vi "Configure Secured TCP Client Certificate and Key.vi"(7 "Client X.509 Certificate":path, 8 "error in (no error)":errorcluster, 9 "password":string, 10 "Client Private Key":path, 11 "Connection.TCP-TLS in":refnum<class "Connection.TCP-TLS.lvclass">) -> (0 "error out":errorcluster, 2 "Auth Client?":bool, 3 "Connection.TCP-TLS out":refnum<class "Connection.TCP-TLS.lvclass">)   [LabVIEW 2020, in "Connection.TCP-TLS.lvclass"]
uses:
  Connection.TCP-TLS.lvclass
  Connection.TCP-TLS.lvclass/Connection.TCP-TLS.ctl
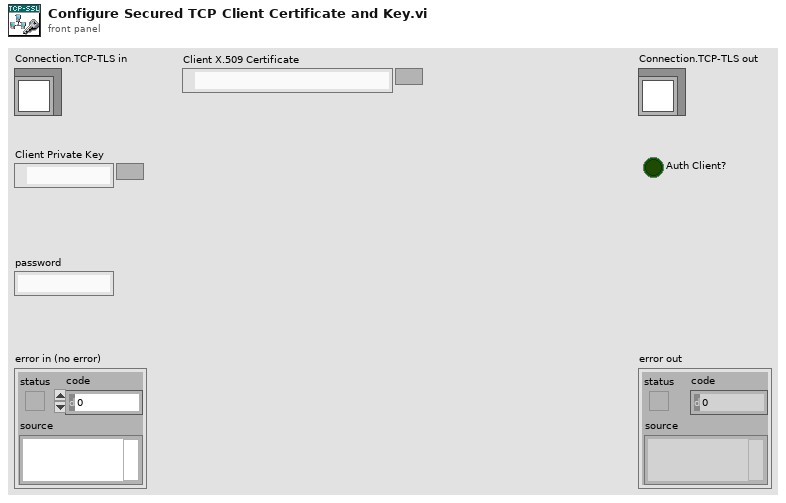
[diagram p1: front panel]
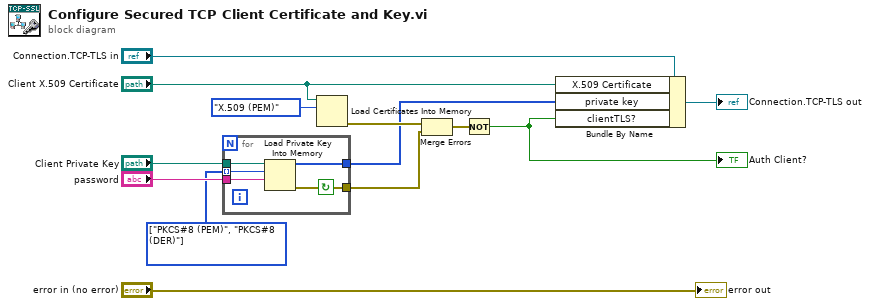
[diagram p0: block diagram]
diagram:
  w4 = enum32{"PKCS#8 (PEM)", "PKCS#8 (DER)"}[] [enum."PKCS#8 (PEM)", enum."PKCS#8 (DER)"] items=["PKCS#8 (PEM)", "PKCS#8 (DER)"]
  n1 = for {
    tunnel: "Client Private Key" -> [w18]
    tunnel: "password" -> [w17]
    tunnel: w4 -> [w16] mode=indexing
    tunnel: [w15] -> w2
    tunnel: [w14] -> w3
    stop <- w14 continue-if-true
    n2 = Load Private Key Into Memory(9:w17, 10:w16, 11:w18) -> (0:w14:errorcluster, 3:w15:u8[])  [unwired: 1 in]
  }
  n3 = Load Certificates Into Memory(10:enum32{"X.509 (PEM)"}."X.509 (PEM)" ("format"), 11:"Client X.509 Certificate") -> (0:w5:errorcluster)  [unwired: 1 in, 1 out]
  n4 = Merge Errors(w5, w3) -> (w6:errorcluster)
  n5 = Not(x=w6) -> (.not. x?=w1:bool)
  "Auth Client?" <- w1
  n6 = Bundle By Name(cluster="Connection.TCP-TLS in", "X.509 Certificate"="Client X.509 Certificate", "private key"=w2, "clientTLS?"=w1) -> (→"Connection.TCP-TLS out":refnum<class "Connection.TCP-TLS.lvclass">)
  "error out" <- "error in (no error)"
